vi "thermal_1.vi"() -> ()   [LabVIEW 2025]
panel:
  out "Thermal Loop Speed (ms)":u32
  out "Thermal Preview":T1(plugin-control)
  in  "Stop Preview":bool
  in  "STOP ACQUISITION":bool
  in  "Focus":dbl(slide) scale=0.0..100.0
  out "Thermal Frame Out":string
  in  "Output Folder":path
  in  "Flag Button":bool
  in  "Stop & Save":bool
  in  "Record":bool
  # "(Enter \"28\")"
  # "Thermal Record"
  # "^ append to base data folder \"...\\test_n\\raw\" for nth recording"
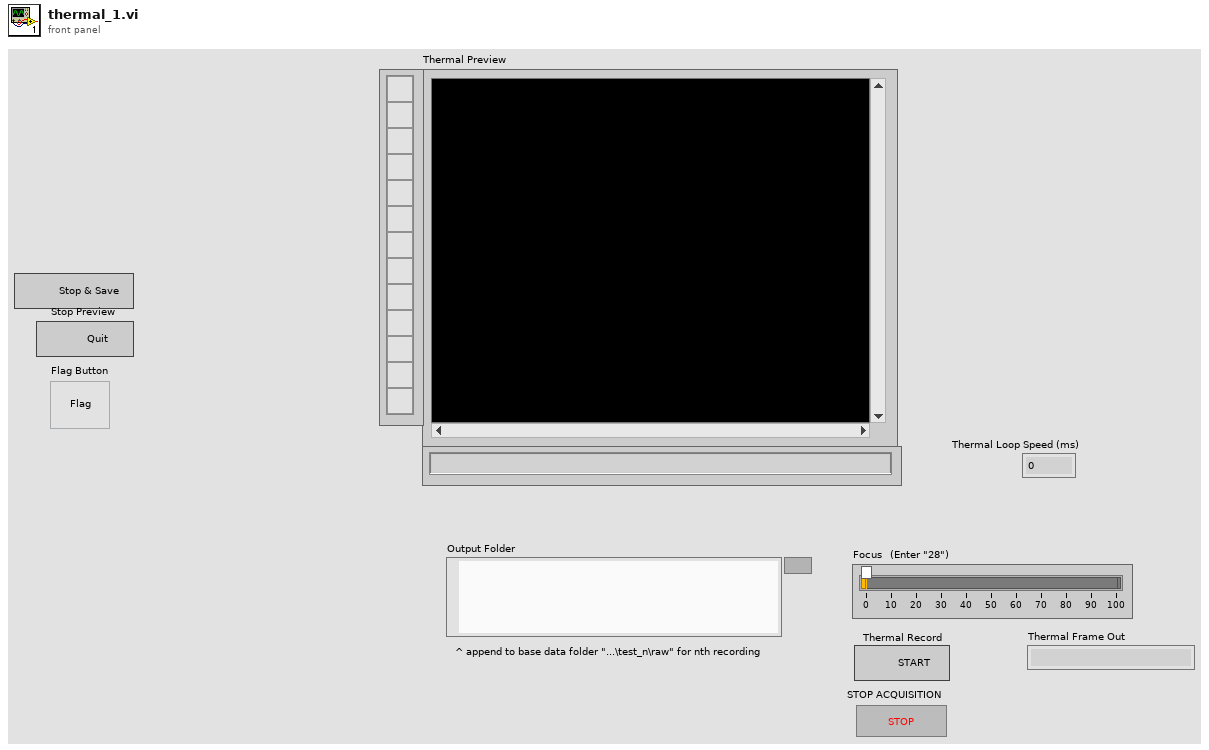
[diagram p1: front panel]
types:
  T1 = typedef "IMAQ Image.ctl" = refnum<image>
  T2 = enum16{"open", "replace", "create", "open or create", "replace or create", "replace or create with confirmation"}
  T3 = enum16{"big-endian, network order", "native, host order", "little-endian"}
  T4 = typedef "Image Type" = u32
  T5 = enum16{"Standard", "Buffered", "CRLF", "Immediate"}
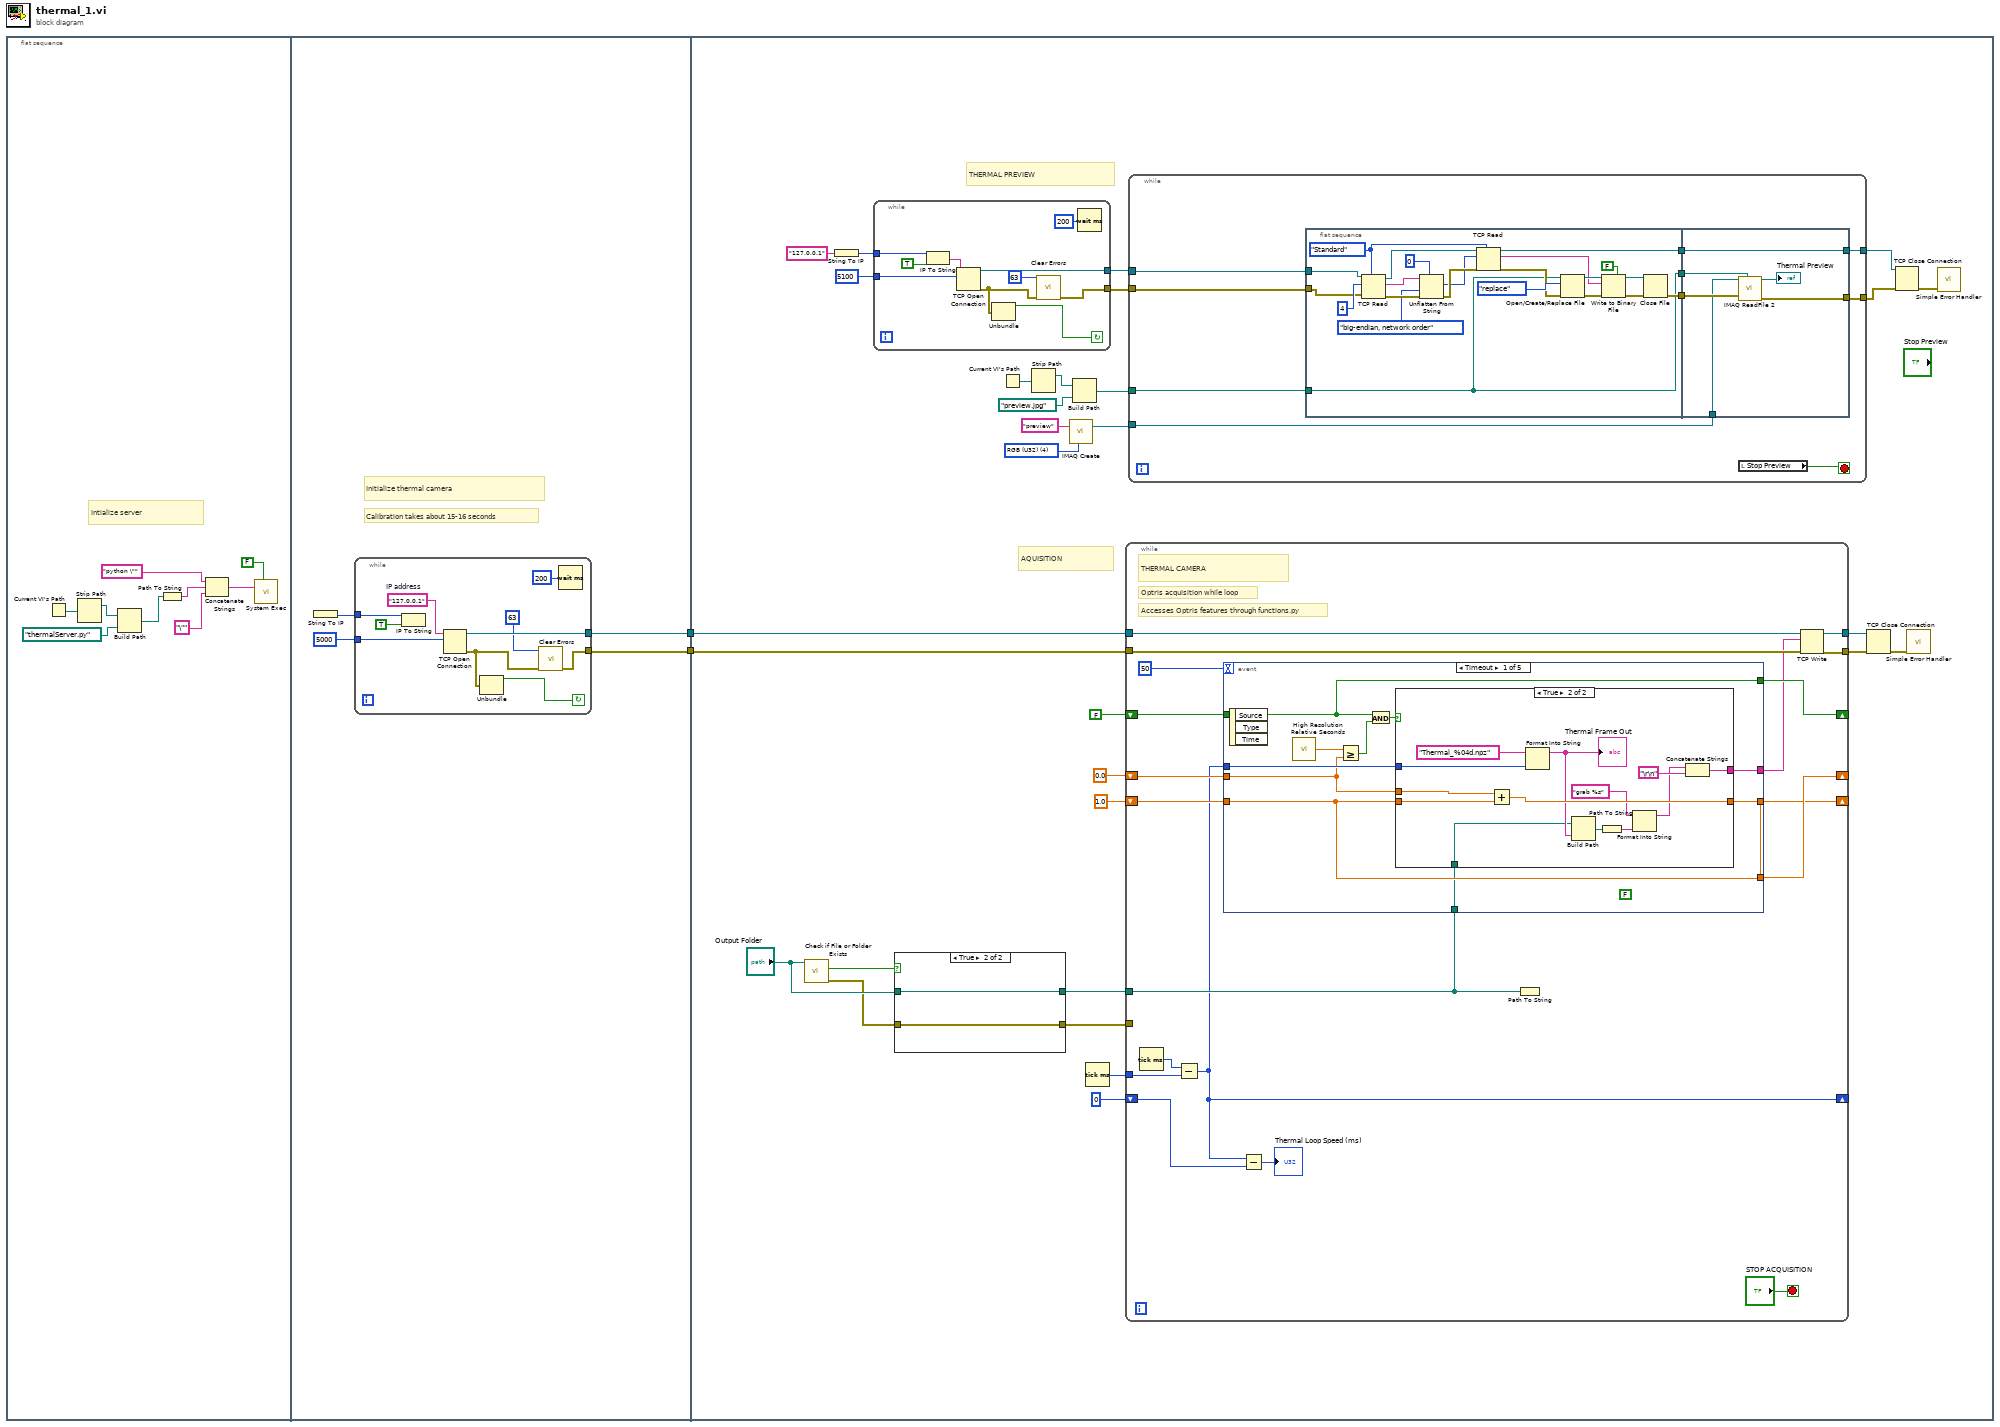
[diagram p0: block diagram]
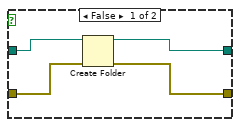
[diagram p2: hidden frame]
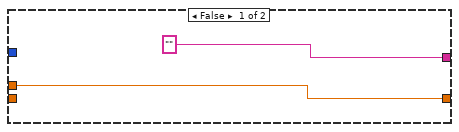
[diagram p3: hidden frame]
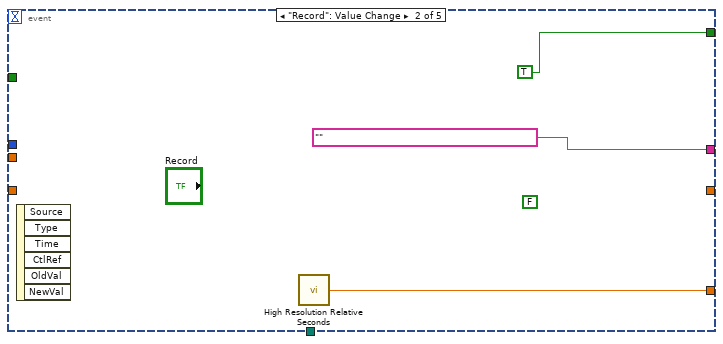
[diagram p4: hidden frame]
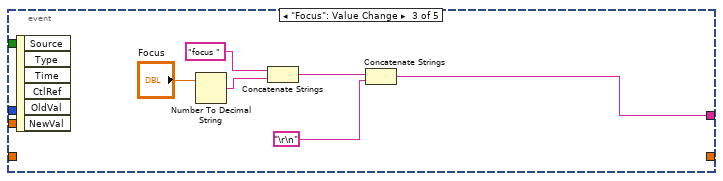
[diagram p5: hidden frame]
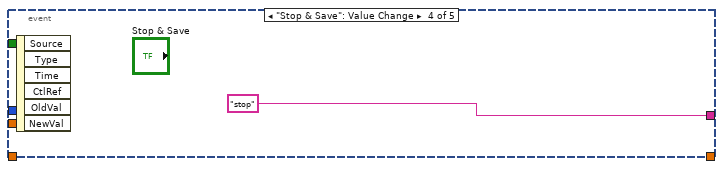
[diagram p6: hidden frame]
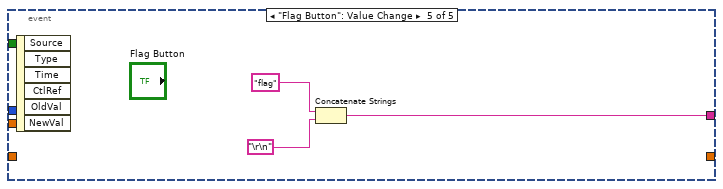
[diagram p7: hidden frame]
diagram:
  n1 = flat-sequence {
    tunnel: [w13] -> w2
    tunnel: [w12] -> w1
    tunnel: w1 -> [w52]
    tunnel: w2 -> [w51]
    frame #0 {
      # "Intialize server"
      n2 = Current VI's Path() -> (path=w6:path)
      n3 = Strip Path(path=w6) -> (stripped path=w7:path)  [unwired: 1 out]
      n4 = Build Path(base path=w7, name or relative path=path "thermalServer.py") -> (appended path=w4:path)
      n5 = Path To String(path=w4) -> (string=w10:string)
      n6 = Concatenate Strings("python \"" ("string"), w10, "\"" ("string")) -> (w9:string)
      n7 = call <vilib>:"System Exec.vi"("wait until completion? (T)"=FALSE, "command line"=w9) -> ()  [unwired: 6 in, 4 out]
    }
    frame #1 {
      # "Initialize thermal camera"
      # "Calibration takes about 15-16 seconds"
      n8 = String To IP() -> (0:w15:u32)  [unwired: 1 in]
      n9 = while {
        tunnel: [w20] -> w13
        tunnel: [w25] -> w12
        tunnel: w15 -> [w24]
        tunnel: u16 5000 ("remote port or service name") -> [w22]
        stop <- w17 continue-if-true
        w16 = "127.0.0.1"  # IP address
        n10 = IP To String(1:TRUE ("dot notation? (F)"), 2:w24) -> ()  [unwired: 1 out]
        n11 = TCP Open Connection(address=w16, remote port or service name=w22) -> (connection ID=w25:refnum<k5>, error out=w21:errorcluster)  [unwired: 3 in]
        n12 = Unbundle(w21) -> ("status"=w17:bool)  [unwired: 2 out]
        n13 = call <vilib>:"Clear Errors.vi"("error in (no error)"=w21, "specific error code to clear (0: all)"=63) -> ("error out"=w20:errorcluster)  [unwired: 4 in, 1 out]
        n14 = Wait (ms)(milliseconds to wait=u32 200) -> ()  [unwired: 1 out]
      }
    }
    frame #2 {
      w36 = T4 4 items=["Grayscale (U8)", "Grayscale (I16)", "Grayscale (SGL)", "Complex (CSG)", "RGB (U32)", "HSL (U32)", "RGB (U64)", "Grayscale (U16)"] ("Image Type")
      # "THERMAL PREVIEW"
      # "AQUISITION"
      n15 = call <vilib>:"Check if File or Folder Exists.vi"("path"="Output Folder") -> ("error out"=w27:errorcluster, "file or folder exists?"=w30:bool)  [unwired: 8 in, 1 out]
      n16 = String To IP(1:"127.0.0.1" ("name")) -> (0:w35:u32)
      n17 = while {
        tunnel: w35 -> [w71]
        tunnel: [w65] -> w34
        tunnel: [w69] -> w33
        tunnel: u16 5100 ("remote port or service name") -> [w67]
        stop <- w62 continue-if-true
        n18 = IP To String(1:TRUE ("dot notation? (F)"), 2:w71) -> (0:w70:string)
        n19 = TCP Open Connection(address=w70, remote port or service name=w67) -> (connection ID=w69:refnum<k5>, error out=w66:errorcluster)  [unwired: 3 in]
        n20 = Unbundle(w66) -> ("status"=w62:bool)  [unwired: 2 out]
        n21 = call <vilib>:"Clear Errors.vi"("error in (no error)"=w66, "specific error code to clear (0: all)"=63) -> ("error out"=w65:errorcluster)  [unwired: 4 in, 1 out]
        n22 = Wait (ms)(milliseconds to wait=u32 200) -> ()  [unwired: 1 out]
      }
      n23 = case shown="True" w30 {
        tunnel: "Output Folder" -> [w59 w61]
        tunnel: [w58 w61] -> w28
        tunnel: w27 -> [w57 w60]
        tunnel: [w56 w60] -> w26
        frame False {
          n24 = Create Folder(path (use dialog)=w59, error in=w57) -> (created path=w58:path, error out=w56:errorcluster)  [unwired: 1 in, 1 out]
        }
        frame True {
        }
      }
      n25 = Current VI's Path() -> (path=w44:path)
      n26 = Strip Path(path=w44) -> (stripped path=w45:path)  [unwired: 1 out]
      n27 = call "IMAQ Create"("Image Name"="preview", "Image Type"=w36) -> ("New Image"=w40:T1)  [unwired: 3 in, 1 out]
      n28 = Build Path(base path=w45, name or relative path=path "preview.jpg") -> (appended path=w43:path)
      n29 = Tick Count (ms)() -> (millisecond timer value=w47:u32)
      n30 = while {
        tunnel: [w128] -> w53
        tunnel: [w127] -> w54
        tunnel: w52 -> [w126]
        tunnel: w51 -> [w125]
        shift-right: [w124] -> _
        shift-left: 0.0 -> [w120]
        shift-right: [w121] -> _
        shift-left: 1.0 -> [w118]
        shift-right: [w122] -> _
        shift-left: FALSE -> [w119]
        tunnel: w47 -> [w114]
        shift-right: [w111] -> _
        shift-left: u32 0 -> [w110]
        tunnel: w28 -> [w113]
        tunnel: w26 -> [_]
        stop <- "STOP ACQUISITION" stop-if-true
        # "THERMAL CAMERA"
        # "Optris acquisition while loop"
        # "Accesses Optris features through functions.py"
        n31 = Tick Count (ms)() -> (millisecond timer value=w115:u32)
        n32 = Subtract(x=w115, y=w114) -> (x-y=w111:u32)
        n33 = event shown="[0] Timeout" {
          selector: _ -> [_ _ _ _ _]
          dyn-events: _ -> [_ _ _ _ _]
          timeout: 50 -> [_ _ _ _ _]
          tunnel: [w134 "" w157 "stop" w166] -> w117
          tunnel: w111 -> [w135 _ _ _ _]
          tunnel: [w132 w156 _ _ _] -> w124
          tunnel: [w130 TRUE _ _ _] -> w122
          tunnel: [w131 _ _ _ _] -> w121
          tunnel: w120 -> [w133 _ _ _ _]
          tunnel: w119 -> [w130 _ _ _ _]
          tunnel: w118 -> [w131 _ _ _ _]
          tunnel: w113 -> [w129 _ _ _ _]
          event Timeout {
            (unwired) FALSE
            n34 = event-data() -> ()  [unwired: 1 in, 3 out]
            n35 = call <vilib>:"High Resolution Relative Seconds.vi"() -> ("relative seconds"=w138:dbl)
            n36 = Greater Or Equal?(x=w138, y=w133) -> (x >= y?=w137:bool)
            n37 = And(x=w130, y=w137) -> (x .and. y?=w136:bool)
            n38 = case shown="True" w136 {
              tunnel: w135 -> [_ w151]
              tunnel: ["" w152] -> w134
              tunnel: w133 -> [w139 w150]
              tunnel: w131 -> [_ w149]
              tunnel: [w139 w148] -> w132
              tunnel: w129 -> [_ w141]
              frame False {
              }
              frame True {
                n39 = Add(x=w150, y=w149) -> (x+y=w148:dbl)
                n40 = Format Into String(format string="Thermal_%04d.npz", w151) -> (resulting string=w142:string)  [unwired: 2 in, 1 out]
                "Thermal Frame Out" <- w142
                n41 = Build Path(base path=w141, name or relative path=w142) -> (appended path=w146:path)
                n42 = Path To String(path=w146) -> (string=w144:string)
                n43 = Format Into String(format string="grab %s", w144) -> (resulting string=w143:string)  [unwired: 2 in, 1 out]
                n44 = Concatenate Strings(w143, "\r\n") -> (w152:string)
              }
            }
          }
          event "Record": Value Change {
            (unwired) FALSE
            n45 = event-data() -> ()  [unwired: 1 in, 6 out]
            n46 = call <vilib>:"High Resolution Relative Seconds.vi"() -> ("relative seconds"=w156:dbl)
          }
          event "Focus": Value Change {
            n47 = event-data() -> ()  [unwired: 1 in, 6 out]
            n48 = Number To Decimal String(number="Focus") -> (decimal integer string=w162:string)  [unwired: 1 in]
            n49 = Concatenate Strings("focus ", w162) -> (w159:string)
            n50 = Concatenate Strings(w159, "\r\n") -> (w157:string)
          }
          event "Stop & Save": Value Change {
            n51 = event-data() -> ()  [unwired: 1 in, 6 out]
          }
          event "Flag Button": Value Change {
            n52 = event-data() -> ()  [unwired: 1 in, 6 out]
            n53 = Concatenate Strings("flag", "\r\n") -> (w166:string)
          }
        }
        n54 = Subtract(x=w111, y=w110) -> (x-y=→"Thermal Loop Speed (ms)":u32)
        n55 = Path To String(path=w113) -> ()  [unwired: 1 out]
        n56 = TCP Write(connection ID=w126, data in=w117, error in (no error)=w125) -> (connection ID out=w127:refnum<k5>, error out=w128:errorcluster)  [unwired: 1 in, 1 out]
      }
      n57 = while {
        tunnel: w40 -> [w76]
        tunnel: [w77] -> w41
        tunnel: [w81] -> w42
        tunnel: w43 -> [w79]
        tunnel: w34 -> [w74]
        tunnel: w33 -> [w73]
        stop <- w72 stop-if-true
        n58 = flat-sequence {
          tunnel: w79 -> [w85]
          tunnel: [w87] -> w80
          tunnel: [w86] -> w78
          tunnel: [w85] -> w75
          tunnel: w74 -> [w83]
          tunnel: w73 -> [w82]
          tunnel: [w109] -> w81
          tunnel: w80 -> [w109]
          tunnel: w78 -> [w108]
          tunnel: [w107] -> w77
          tunnel: w76 -> [w106]
          tunnel: w75 -> [w105]
          frame #0 {
            w96 = T5."Standard" ("mode (standard)")
            n59 = TCP Read(connection ID=w82, bytes to read=4, error in (no error)=w83, 7:w96) -> (connection ID out=w99:refnum<k5>, data out=w84:string, error out=w102:errorcluster)  [unwired: 1 in]
            n60 = Unflatten From String(type=0, binary string=w84, byte order (0:big-endian, network order)=T3."big-endian, network order", error in (no error)=w102) -> (value=w97:i32, error out=w98:errorcluster)  [unwired: 1 in, 1 out]
            n61 = TCP Read(connection ID=w99, bytes to read=w97, error in (no error)=w98, 7:w96) -> (connection ID out=w87:refnum<k5>, data out=w92:string, error out=w94:errorcluster)  [unwired: 1 in]
            n62 = Open/Create/Replace File(file path (use dialog)=w85, error in=w94, operation (0:open)=T2."replace") -> (refnum out=w93:refnum<file>, error out=w90:errorcluster)  [unwired: 3 in, 1 out]
            n63 = Write to Binary File(file (use dialog)=w93, data=w92, error in=w90, 5:FALSE ("prepend array or string size? (T)")) -> (refnum out=w88:refnum<file>, error out=w89:errorcluster)  [unwired: 2 in, 1 out]
            n64 = Close File(refnum=w88, error in=w89) -> (error out=w86:errorcluster)  [unwired: 1 out]
          }
          frame #1 {
            n65 = call "IMAQ ReadFile 2"("File Path"=w105, "error in (no error)"=w108, "Image"=w106) -> ("error out"=w107:errorcluster, "Image Out"=→"Thermal Preview":T1)  [unwired: 4 in, 3 out]
          }
        }
        n66 = local read "Stop Preview"() -> (w72:bool)
      }
      n67 = TCP Close Connection(connection ID=w54, error in (no error)=w53) -> (error out=w55:errorcluster)  [unwired: 1 in, 1 out]
      n68 = TCP Close Connection(connection ID=w42, error in (no error)=w41) -> (error out=w39:errorcluster)  [unwired: 1 in, 1 out]
      n69 = call <vilib>:"Simple Error Handler.vi"("error in (no error)"=w55) -> ()  [unwired: 4 in, 5 out]
      n70 = call <vilib>:"Simple Error Handler.vi"("error in (no error)"=w39) -> ()  [unwired: 4 in, 5 out]
    }
  }
